vi "Device Worker.vi"(8 "error in":errorcluster, 10 "Session":T3, 11 "transport config":T1) -> (0 "error out":errorcluster)   [LabVIEW 2015, in "Lengmur_socket.lvlib"]
uses:
  Lengmur_socket.lvlib
  Types/Responses/Telemetry Response.ctl
  Types/Measurement Point.ctl
  Types/Device Config.ctl
  Types/Device Event.ctl
  Types/Device  Operation.ctl
  Types/Responses/Get Response.ctl
  Device Command.ctl
  Types/Device Session.ctl
  Types/Transport Config.ctl
  Types/Transport Kind.ctl
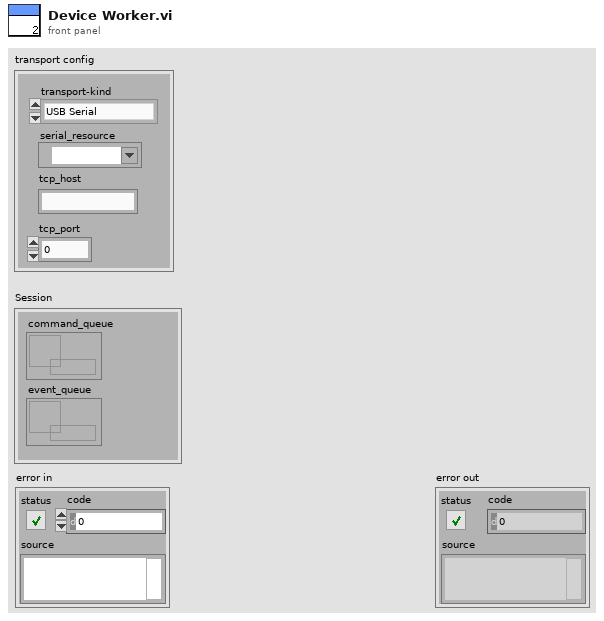
[diagram p1: front panel]
types:
  T1 = typedef "Lengmur_socket.lvlib/Transport Config.ctl" = cluster{"transport-kind":T2, "serial_resource":refnum<visa-resource-name>, "tcp_host":string, "tcp_port":u16}
  T2 = typedef "Lengmur_socket.lvlib/Transport Kind.ctl" = enum16{"USB Serial", "Ethernet TCP"}
  T3 = typedef "Lengmur_socket.lvlib/Device Session.ctl" = cluster{"command_queue":refnum<queue>, "event_queue":refnum<queue>}
  T4 = typedef "Lengmur_socket.lvlib/Device  Operation.ctl" = enum16{"Get Configuration", "Set Configuration", "Start Sweep", "Shutdown"}
  T5 = enum16{"None", "Telemetry", "Command Response", "Sweep Complete", "Device Error", "Transport Error"}
  T6 = typedef "Lengmur_socket.lvlib/Device Event.ctl" = cluster{"event_type":enum16{"None", "Telemetry", "Command Response", "Sweep Complete", "Device Error", "Transport Error"}, "measurement":T7, "configuration":T8, "sweep_points":T7[], "command_ok":bool, "device_error":string, "error":errorcluster}
  T7 = typedef "Lengmur_socket.lvlib/Measurement Point.ctl" = cluster{"voltage_code":i16, "current_code":i16}
  T8 = typedef "Lengmur_socket.lvlib/Device Config.ctl" = cluster{"sample_rate":i32, "min_voltage":i32, "max_voltage":i32, "shunt_res":i32}
  T9 = typedef "Lengmur_socket.lvlib/Get Response.ctl" = cluster{"type":string, "ok":bool, "device_config":T8}
  T10 = typedef "Lengmur_socket.lvlib/Telemetry Response.ctl" = cluster{"type":string, "voltage":i16, "current":i16}
  T11 = cluster{"transport_kind":T2, "visa_session":refnum<visa-resource-name>, "tcp_session":refnum<k5>}
  T12 = typedef "Lengmur_socket.lvlib/Decoded Frame.ctl" = cluster{"packet_type":u8, "payload":string}
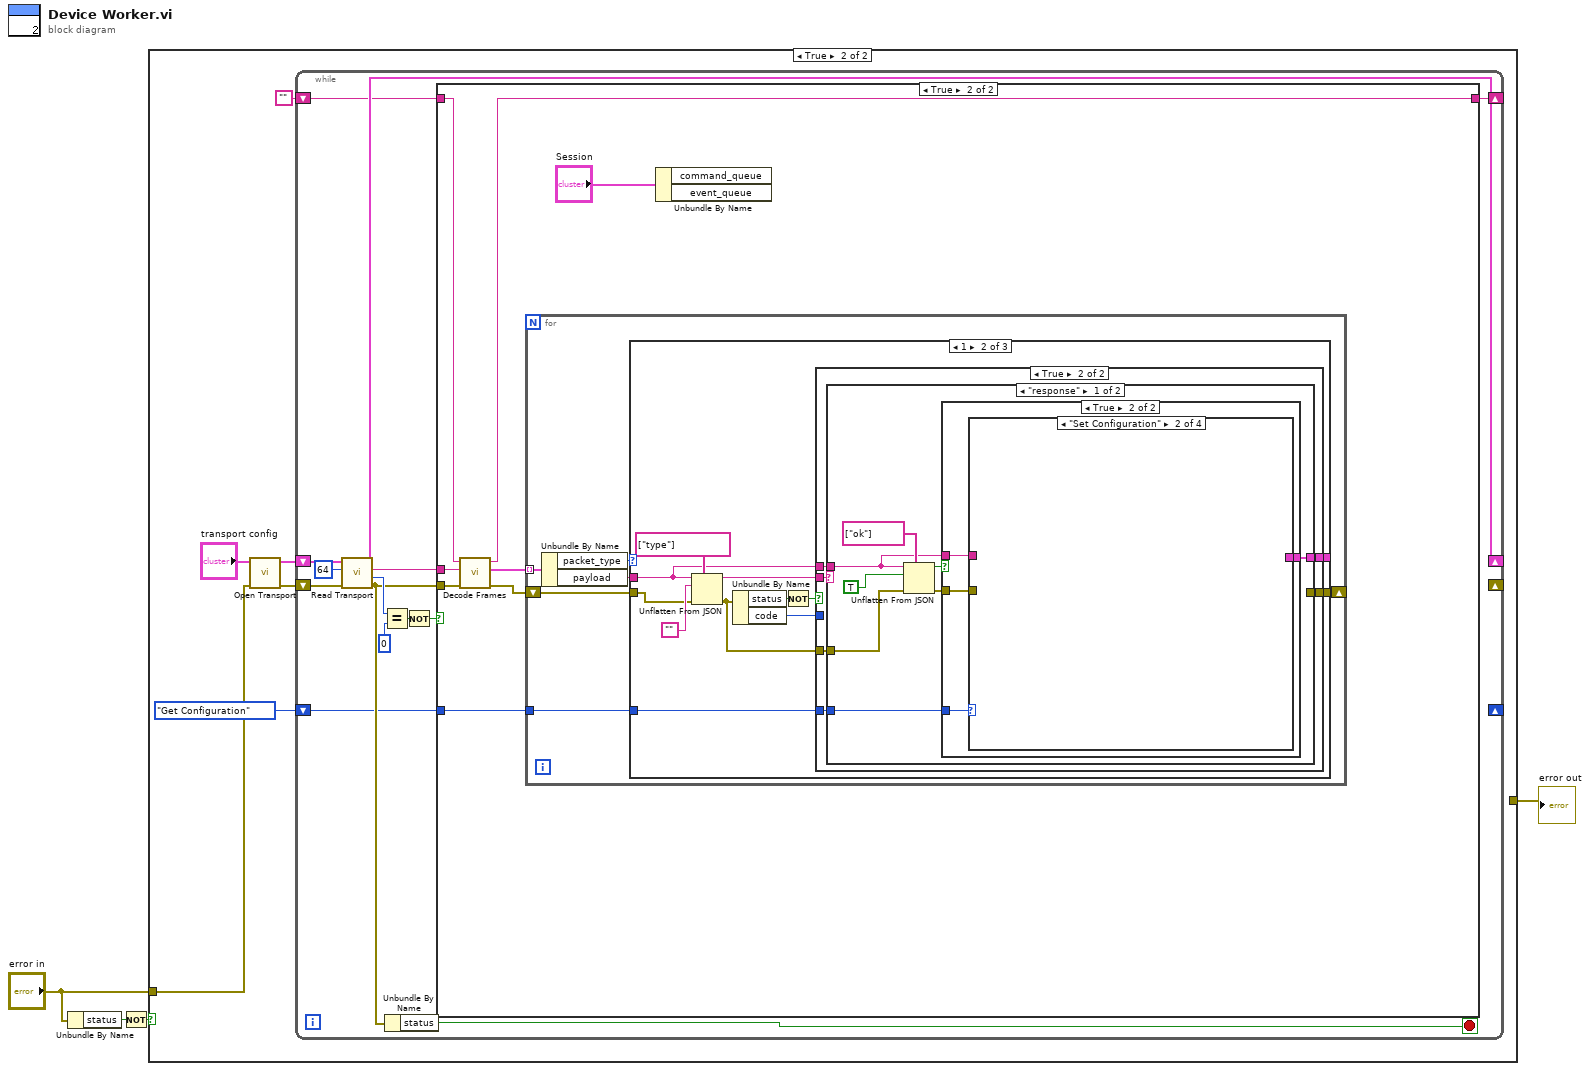
[diagram p0: block diagram]
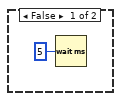
[diagram p3: hidden frame]
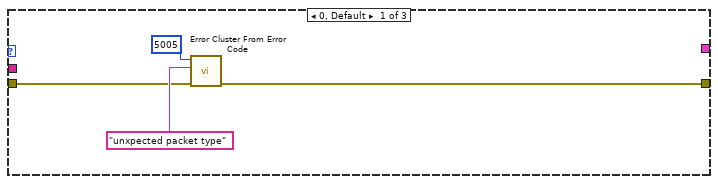
[diagram p4: hidden frame]
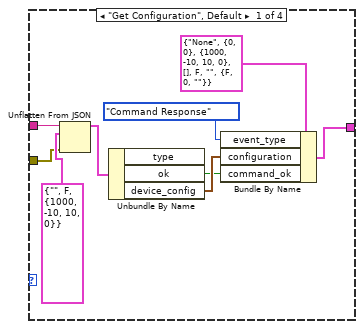
[diagram p7: hidden frame]
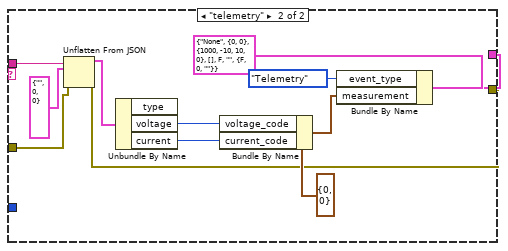
[diagram p10: hidden frame]
diagram:
  n1 = Unbundle By Name("error in") -> ("status"=w3:bool)
  n2 = Not(x=w3) -> (.not. x?=w2:bool)
  n3 = case shown="True" w2 {
    tunnel: "error in" -> [w5 w11]
    tunnel: [w5 _] -> w1
    frame False {
    }
    frame True {
      n4 = call "Open Transport.vi"("error in"=w11, "transport config"="transport config") -> ("error out"=w9:errorcluster, "transport session"=w10:T11)  [unwired: 8 in]
      n5 = while {
        shift-right: [w15] -> _
        shift-left: "" -> [w19]
        shift-right: [w24] -> _
        shift-left: w10 -> [w25]
        shift-right: _ -> [_]
        shift-left: w9 -> [w23]
        shift-right: _ -> [_]
        shift-left: Device__Operation."Get Configuration" ("operation") -> [w12]
        stop <- w13 stop-if-true
        n6 = call "Read Transport.vi"("error in"=w23, "max bytes"=u32 64, "transport session"=w25) -> ("error out"=w14:errorcluster, "bytes read"=w21:u32, "data out"=w18:string, "transport session out"=w24:T11)  [unwired: 5 in]
        n7 = Equal?(x=w21, y=u32 0) -> (x = y?=w16:bool)
        n8 = Unbundle By Name(w14) -> ("status"=w13:bool)
        n9 = Not(x=w16) -> (.not. x?=w17:bool)
        n10 = case shown="True" w17 {
          tunnel: w19 -> [_ w34]
          tunnel: w18 -> [_ w33]
          tunnel: w14 -> [_ w32]
          tunnel: [_ w31] -> w15
          tunnel: w12 -> [_ w27]
          frame False {
            n11 = Wait (ms)(milliseconds to wait=u32 5) -> ()  [unwired: 1 out]
          }
          frame True {
            n12 = call "Decode Frames.vi"("error in"=w32, "data in"=w33, "pending bytes"=w34) -> ("error out"=w28:errorcluster, "decoded frames"=w30:T12[], "remaining bytes"=w31:string)  [unwired: 6 in]
            n13 = for {
              tunnel: w30 -> [w40] mode=indexing
              shift-right: [w37] -> _
              shift-left: w28 -> [w38]
              tunnel: w27 -> [w35]
              n14 = Unbundle By Name(w40) -> ("packet_type"=w39:u8, "payload"=w36:string)
              n15 = case shown="1" w39 {
                tunnel: w38 -> [w42 w54 _]
                tunnel: [w41 w45 _] -> w37
                tunnel: w36 -> [_ w49 _]
                tunnel: [_ w48 _] -> _
                tunnel: w35 -> [_ w47 _]
                frame 0, Default {
                  n16 = call <vilib>:"Error Cluster From Error Code.vi"("error in (no error)"=w42, "error message (\"\")"="unxpected packet type" ("error message (\"\")"), "error code (0)"=5005) -> ("error out"=w41:errorcluster)  [unwired: 6 in]
                }
                frame 1 {
                  n17 = Unflatten From JSON(path=string[] ["type"], JSON string=w49, type and defaults="", error in (no error)=w54) -> (value=w50:string, error out=w46:errorcluster)  [unwired: 3 in]
                  n18 = Unbundle By Name(w46) -> ("status"=w53:bool, "code"=w51:i32)
                  n19 = Not(x=w53) -> (.not. x?=w52:bool)
                  n20 = case shown="True" w52 {
                    tunnel: w51 -> [_ _]
                    tunnel: w50 -> [_ w62]
                    tunnel: w49 -> [_ w61]
                    tunnel: [_ w60] -> w48
                    tunnel: w47 -> [_ w59]
                    tunnel: w46 -> [_ w58]
                    tunnel: [_ w57] -> w45
                    frame False {
                    }
                    frame True {
                      n21 = case shown="\"response\"" w62 {
                        tunnel: w61 -> [w65 w95]
                        tunnel: [w63 w86] -> w60
                        tunnel: w59 -> [w66 _]
                        tunnel: w58 -> [w69 w85]
                        tunnel: [_ w84] -> w57
                        frame "response" {
                          n22 = Unflatten From JSON(path=string[] ["ok"], JSON string=w65, type and defaults=TRUE, error in (no error)=w69) -> (value=w67:bool, error out=w64:errorcluster)  [unwired: 3 in]
                          n23 = case shown="True" w67 {
                            tunnel: w66 -> [_ w74]
                            tunnel: w65 -> [_ w73]
                            tunnel: w64 -> [_ w72]
                            tunnel: [_ w71] -> w63
                            frame False {
                            }
                            frame True {
                              n24 = case shown="\"Set Configuration\"" w74 {
                                tunnel: w73 -> [w83 _ _ _]
                                tunnel: w72 -> [w81 _ _ _]
                                tunnel: [w75 _ _ _] -> w71
                                frame "Get Configuration", Default {
                                n25 = Unflatten From JSON(JSON string=w83, type and defaults=T9 {"type"="", "ok"=FALSE, "device_config"={"sample_rate"=1000, "min_voltage"=-10, "max_voltage"=10, "shunt_res"=0}} ("payload"), error in (no error)=w81) -> (value=w80:T9)  [unwired: 4 in, 1 out]
                                n26 = Unbundle By Name(w80) -> ("ok"=w76:bool, "device_config"=w78:T8)  [unwired: 1 out]
                                n27 = Bundle By Name(cluster=T6 {"event_type"=enum."None", "measurement"={"voltage_code"=0, "current_code"=0}, "configuration"={"sample_rate"=1000, "min_voltage"=-10, "max_voltage"=10, "shunt_res"=0}, "sweep_points"=[], "command_ok"=FALSE, "device_error"="", "error"={"status"=FALSE, "code"=0, "source"=""}} ("device_event"), "event_type"=T5."Command Response", "configuration"=w78, "command_ok"=w76) -> (w75:T6)
                                }
                                frame "Set Configuration" {
                                }
                                frame "Start Sweep" {
                                }
                                frame "Shutdown" {
                                }
                              }
                            }
                          }
                        }
                        frame "telemetry" {
                          n28 = Unflatten From JSON(JSON string=w95, type and defaults=T10 {"type"="", "voltage"=0, "current"=0} ("payload"), error in (no error)=w85) -> (value=w93:T10, error out=w84:errorcluster)  [unwired: 4 in]
                          n29 = Unbundle By Name(w93) -> ("voltage"=w89:i16, "current"=w88:i16)  [unwired: 1 out]
                          n30 = Bundle By Name(cluster=T7 {"voltage_code"=0, "current_code"=0} ("measurement_point"), "voltage_code"=w89, "current_code"=w88) -> (w87:T7)
                          n31 = Bundle By Name(cluster=T6 {"event_type"=enum."None", "measurement"={"voltage_code"=0, "current_code"=0}, "configuration"={"sample_rate"=1000, "min_voltage"=-10, "max_voltage"=10, "shunt_res"=0}, "sweep_points"=[], "command_ok"=FALSE, "device_error"="", "error"={"status"=FALSE, "code"=0, "source"=""}} ("device_event"), "event_type"=T5."Telemetry", "measurement"=w87) -> (w86:T6)
                        }
                      }
                    }
                  }
                }
                frame 2 {
                }
              }
            }
            n32 = Unbundle By Name("Session") -> ()  [unwired: 2 out]
          }
        }
      }
    }
  }
  "error out" <- w1
